vi "RDV-singleGraph-SelectData.vi"(8 "error in (no error)":errorcluster, 11 "RDV-Reflection_Data_viewer in":refnum<class "RDV-Reflection_Data_viewer.lvclass">) -> (0 "error out":errorcluster, 3 "RDV-Reflection_Data_viewer out":refnum<class "RDV-Reflection_Data_viewer.lvclass">)   [LabVIEW 2020, in "RDV-Reflection_Data_viewer.lvclass"]
doc: "Selects which data the single-graph viewer shows."
uses:
  RDV-Reflection_Data_viewer.lvclass
  RDV-Reflection_Data_viewer.lvclass/RDV-Reflection_Data_viewer.ctl
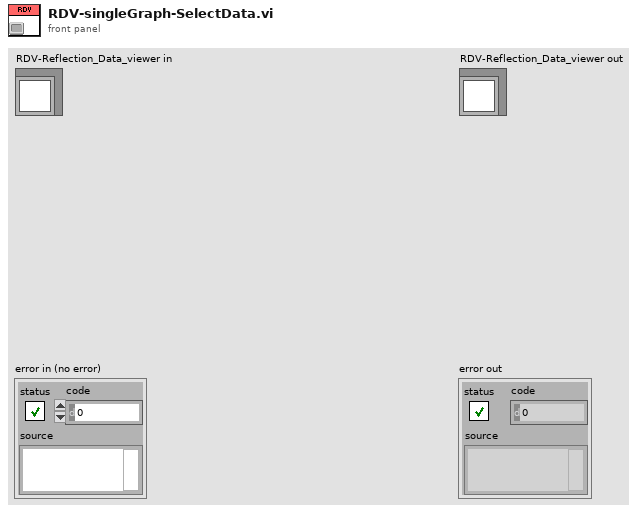
[diagram p1: front panel]
types:
  T1 = cluster{"Frequency":dbl[], "Reflection'":dbl[]}[]
  T2 = cluster{"Frequency":dbl[], "Reflection'":dbl[]}[][]
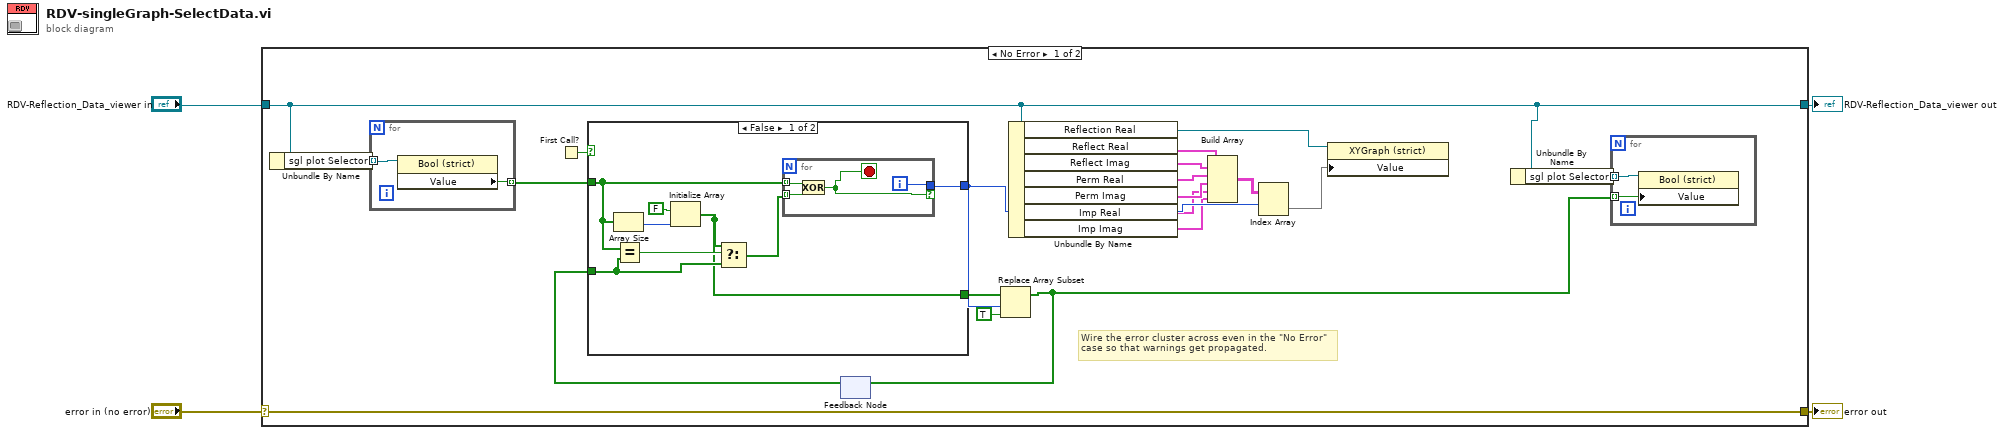
[diagram p0: block diagram]
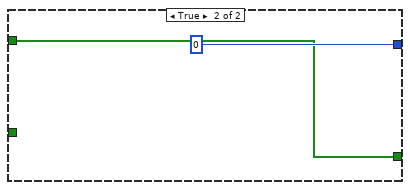
[diagram p2: hidden frame]
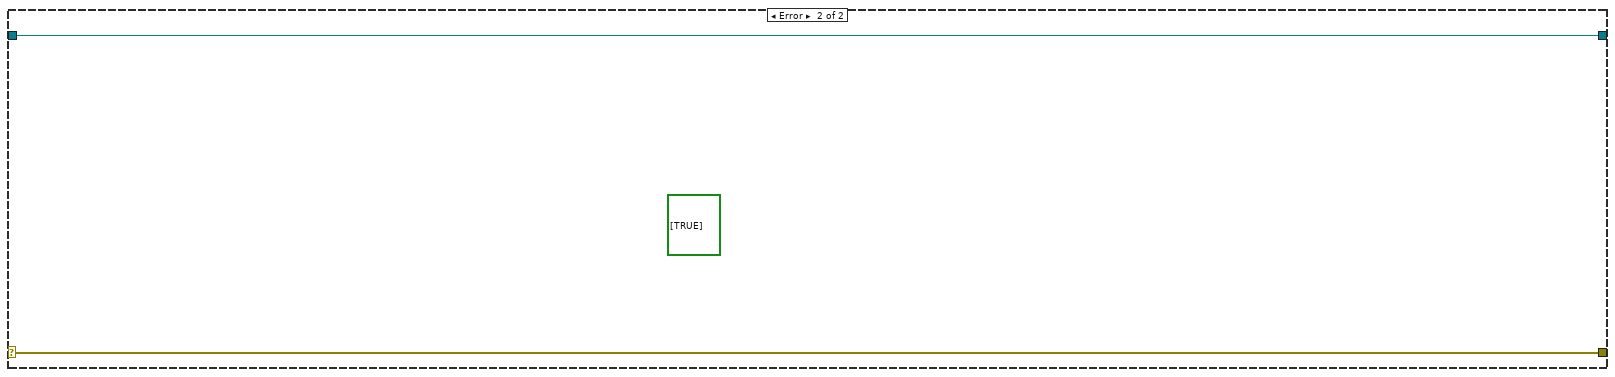
[diagram p3: hidden frame]
diagram:
  n1 = case shown="No Error" "error in (no error)" {
    selector: "error in (no error)" -> [w24 w44]
    tunnel: [w24 w44] -> w3
    tunnel: [w8 w43] -> w1
    tunnel: "RDV-Reflection_Data_viewer in" -> [w8 w43]
    frame No Error {
      # "Wire the error cluster across even in the \"No Error\"\ncase so that warnings get propagated."
      n2 = Unbundle By Name(w8) -> ("sgl plot Selector"=w11:refnum<vi>[])
      n3 = for {
        tunnel: w11 -> [w28] mode=indexing
        tunnel: [w27] -> w10 mode=indexing
        n4 = property on="Property Node" class="Bool (strict)"(reference=w28) -> ("Value"=w27:bool)  [unwired: 1 in, 2 out]
      }
      n5 = First Call?() -> (First Call?: T/F=w13:bool)
      n6 = feedback #1() -> (w12:bool[])  [unwired: 1 in]
      n7 = case shown="False" w13 {
        tunnel: [w30 w41] -> w16
        tunnel: [w34 0] -> w15
        tunnel: w10 -> [w33 w41]
        tunnel: w12 -> [w31 _]
        frame False {
          n8 = Array Size(array=w33) -> (size(s)=w36:i32)
          n9 = Equal?(x=w33, y=w31) -> (x = y?=w32:bool)
          n10 = Initialize Array(FALSE, w36) -> (w30:bool[])
          n11 = Select(t=w30, s=w32, f=w31) -> (s? t:f=w29:bool[])
          n12 = for {
            tunnel: w33 -> [w39] mode=indexing
            tunnel: [w40] -> w34 if=w37
            tunnel: w29 -> [w38] mode=indexing
            i -> [w40]
            stop <- w37 stop-if-true
            n13 = Exclusive Or(1:w38, 2:w39) -> (0:w37:bool)
          }
        }
        frame True {
        }
      }
      n14 = Replace Array Subset(array=w16, new element=TRUE ("new element/subarray"), index=w15) -> (w7:bool[])
      n15 = feedback-in #1(w7) -> ()
      n16 = Unbundle By Name(w8) -> ("Reflection Real"=w19:refnum<vi>, "Reflect Real"=w23:T1, "Reflect Imag"=w22:T1, "Perm Real"=w21:T1, "Perm Imag"=w20:T1, "Imp Real"=w6:T1, "Imp Imag"=w5:T1)
      n17 = Build Array(w23, w22, w21, w20, w6, w5) -> (w18:T2)
      n18 = Index Array(array=w18, index (row)=w15) -> (element=w17:T1)  [unwired: 1 in]
      n19 = property on="Property Node" class="XYGraph (strict)"(reference=w19, "Value"=w17) -> ()  [unwired: 1 in, 2 out]
      n20 = Unbundle By Name(w8) -> ("sgl plot Selector"=w9:refnum<vi>[])
      n21 = for {
        tunnel: w9 -> [w26] mode=indexing
        tunnel: w7 -> [w25] mode=indexing
        n22 = property on="Property Node" class="Bool (strict)"(reference=w26, "Value"=w25) -> ()  [unwired: 1 in, 2 out]
      }
    }
    frame Error {
      (unwired) bool[] [TRUE]
    }
  }
  "error out" <- w3
  "RDV-Reflection_Data_viewer out" <- w1
